vi "over seq vi.vi"(8 "y":i32=30, 11 "Read Seq":string) -> (3 "result seq":string)   [LabVIEW 2018]
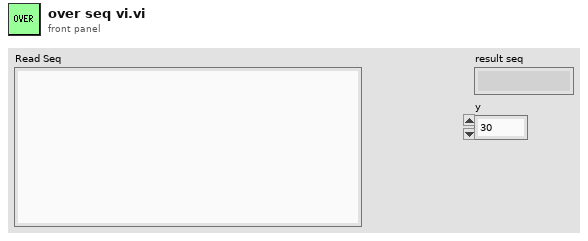
[diagram p1: front panel]
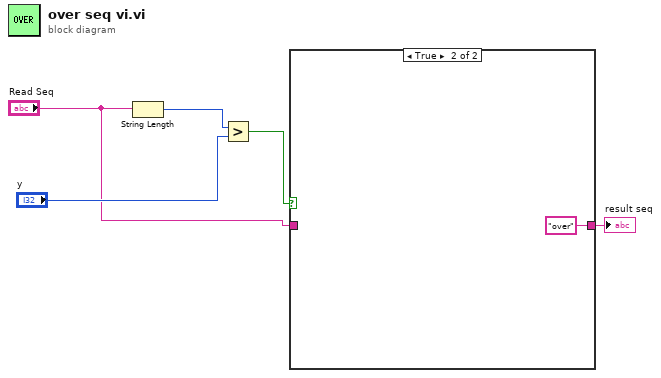
[diagram p0: block diagram]
diagram:
  n1 = String Length(string="Read Seq") -> (length=w5:i32)
  n2 = Greater?(x=w5, y="y") -> (0:w3:bool)
  n3 = case shown="True" w3 {
    tunnel: "Read Seq" -> [w6 _]
    tunnel: [w6 "over" ("Read Seq")] -> w1
    frame False {
    }
    frame True {
    }
  }
  "result seq" <- w1
